vi "eDyno Accel Synth.vi"(0 "Fault Injection":T3={"Imbalance ON"=FALSE, "Imbalance (g)"=0.5, "Misalignment ON"=FALSE, "Misalignment (g)"=0.2, "Bearing BPFO ON"=FALSE, "Bearing Impact (g)"=2.0, "Motor Ripple ON"=FALSE, "Torque Ripple (g)"=0.3, "PWM Noise ON"=FALSE, "PWM Level (g)"=0.05}, 1 "Sim Config":T2={"Sample Rate (Hz)"=51200.0, "Ref Speed (rpm)"=3000.0, "Baseline 1x (g)"=0.02, "Noise Floor (g rms)"=0.01, "BPFO Order"=3.57, "Resonance (Hz)"=3500.0, "Decay (ms)"=0.8, "Pole Pairs"=4.0, "PWM Carrier (Hz)"=16000.0}, 2 "rpm start":dbl=3000.0, 3 "rpm end":dbl=3000.0, 4 "Samples":i32=5120, 5 "State in":cluster{"Shaft Rev":dbl, "Sample Index":dbl}) -> (14 "Accel (g)":dbl[](array[numeric]), 15 "Fault Frequencies (Hz)":T1, 16 "Speed (rpm)":dbl[](array[numeric]), 17 "Tach Pulse 1ppr (0/1)":dbl[](array[numeric]), 19 "State out":cluster{"Shaft Rev":dbl, "Sample Index":dbl})   [LabVIEW 2026]
doc: "Synthesizes one block of eDyno drivetrain acceleration (g) as seen by a PCB 356A15 ICP accelerometer (one axis) on an e-bike motor housing.\n\nSpeed ramps linearly from rpm start to rpm end across the block, and every order tracks speed. Shaft phase (revolutions) and the sample counter travel in State in/State out: feed State out back into State in through a shift register in the caller so consecutive blocks are phase-continuous.\n\nBaseline: a small 1x residual plus broadband noise. Injectable faults (Fault Injection cluster):\n- Imbalance: 1x order, amplitude scales with (rpm/ref)^2\n- Misalignment: 2x order\n- Bearing outer race (BPFO): impacts every 1/(BPFO order x shaft Hz) ringing the housing resonance with exponential decay\n- Motor torque ripple: 6 x pole-pairs order\n- Inverter PWM: carrier with sidebands at carrier +/- 2 x electrical frequency\n\nFault Frequencies returns the expected frequencies at rpm end, for the engineer to check against the spectrum. Speed (rpm) returns the instantaneous shaft speed per sample, and Tach Pulse 1ppr a 50 % duty once-per-rev square wave whose rising edge is at shaft angle 0 - both phase-locked to Accel (g) for order analysis."
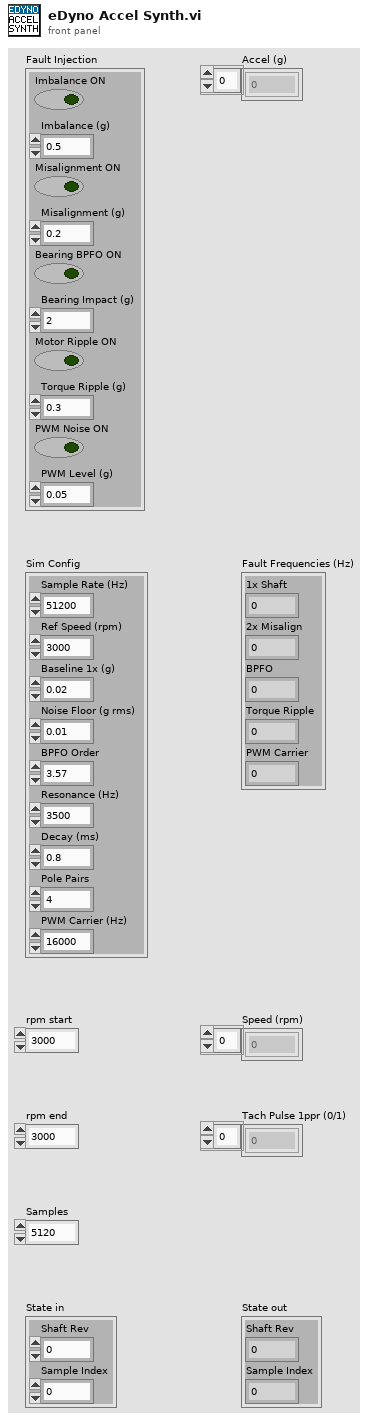
[diagram p1: front panel]
types:
  T1 = cluster{"1x Shaft":dbl, "2x Misalign":dbl, "BPFO":dbl, "Torque Ripple":dbl, "PWM Carrier":dbl}
  T2 = cluster{"Sample Rate (Hz)":dbl, "Ref Speed (rpm)":dbl, "Baseline 1x (g)":dbl, "Noise Floor (g rms)":dbl, "BPFO Order":dbl, "Resonance (Hz)":dbl, "Decay (ms)":dbl, "Pole Pairs":dbl, "PWM Carrier (Hz)":dbl}
  T3 = cluster{"Imbalance ON":bool, "Imbalance (g)":dbl, "Misalignment ON":bool, "Misalignment (g)":dbl, "Bearing BPFO ON":bool, "Bearing Impact (g)":dbl, "Motor Ripple ON":bool, "Torque Ripple (g)":dbl, "PWM Noise ON":bool, "PWM Level (g)":dbl}
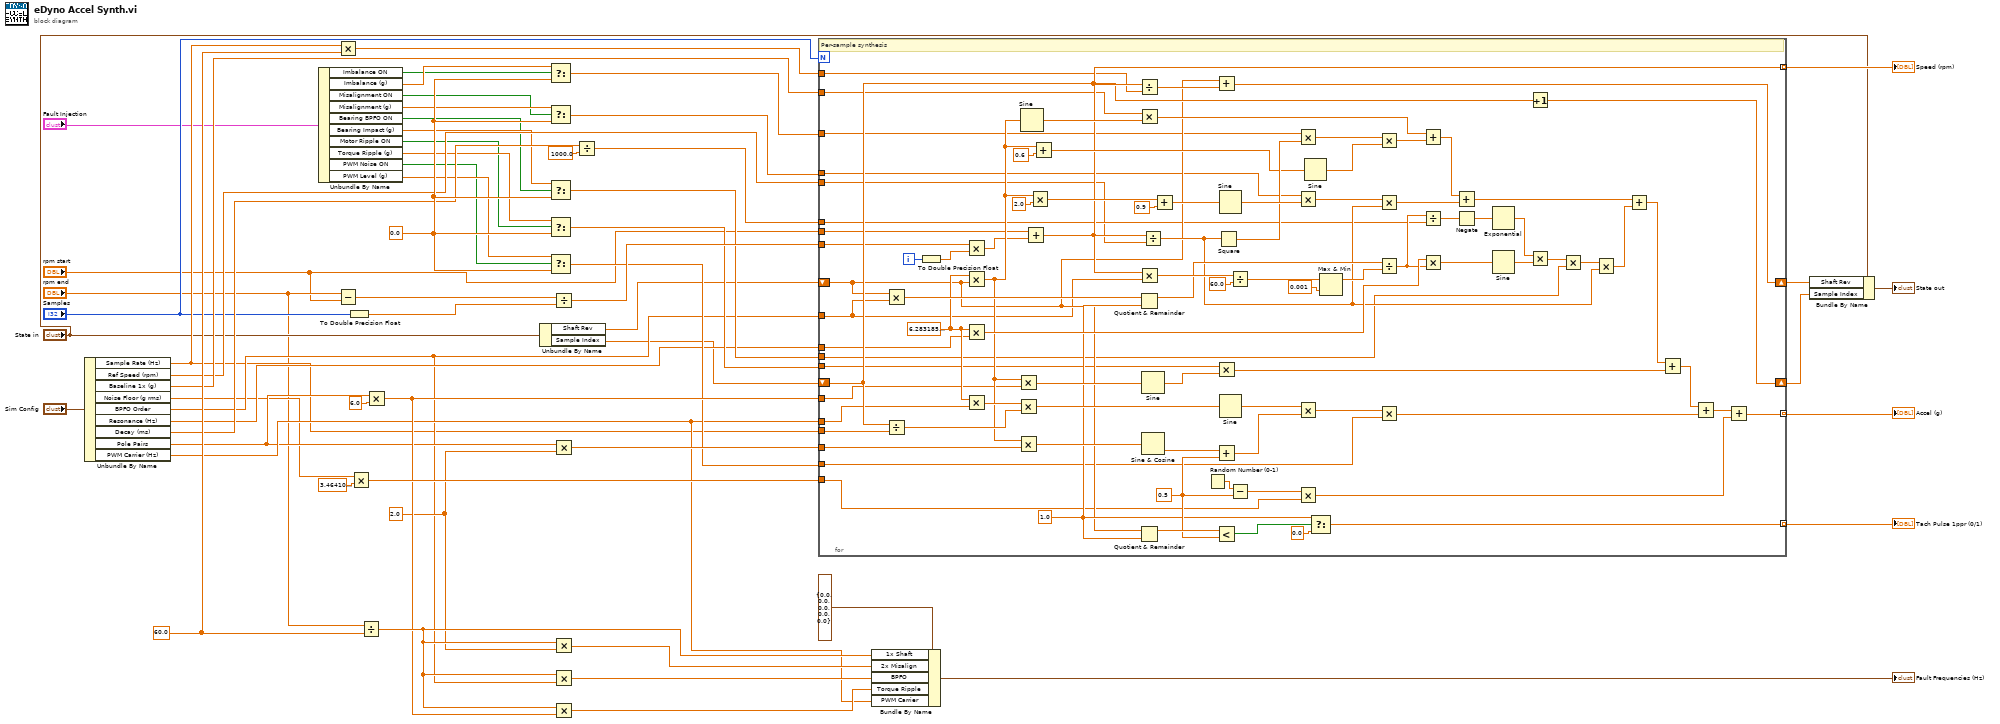
[diagram p0: block diagram]
diagram:
  w39 = 2.0 ("2")
  w36 = 60.0 ("60")
  w35 = 0.0 ("zero")
  n1 = Unbundle By Name("Sim Config") -> ("Sample Rate (Hz)"=w26:dbl, "Ref Speed (rpm)"=w27:dbl, "Baseline 1x (g)"=w28:dbl, "Noise Floor (g rms)"=w29:dbl, "BPFO Order"=w30:dbl, "Resonance (Hz)"=w31:dbl, "Decay (ms)"=w32:dbl, "Pole Pairs"=w33:dbl, "PWM Carrier (Hz)"=w34:dbl)
  n2 = Unbundle By Name("Fault Injection") -> ("Imbalance ON"=w16:bool, "Imbalance (g)"=w17:dbl, "Misalignment ON"=w18:bool, "Misalignment (g)"=w19:dbl, "Bearing BPFO ON"=w20:bool, "Bearing Impact (g)"=w21:dbl, "Motor Ripple ON"=w22:bool, "Torque Ripple (g)"=w23:dbl, "PWM Noise ON"=w24:bool, "PWM Level (g)"=w25:dbl)
  n3 = Multiply(x=w26, y=w36) -> (x*y=w49:dbl)
  n4 = Subtract(x="rpm end", y="rpm start") -> (x-y=w47:dbl)
  n5 = To Double Precision Float(number="Samples") -> (double precision float=w46:dbl)
  n6 = Multiply(x=w29, y=3.4641016151377544 ("sqrt12")) -> (x*y=w53:dbl)
  n7 = Divide(x="rpm end", y=w36) -> (x/y=w54:dbl)
  n8 = Multiply(x=w33, y=6.0 ("6")) -> (x*y=w51:dbl)
  n9 = Unbundle By Name("State in") -> ("Shaft Rev"=w12:dbl, "Sample Index"=w13:dbl)
  n10 = Select(t=w17, s=w16, f=w35) -> (s? t:f=w41:dbl)
  n11 = Select(t=w19, s=w18, f=w35) -> (s? t:f=w42:dbl)
  n12 = Select(t=w21, s=w20, f=w35) -> (s? t:f=w43:dbl)
  n13 = Select(t=w23, s=w22, f=w35) -> (s? t:f=w44:dbl)
  n14 = Select(t=w25, s=w24, f=w35) -> (s? t:f=w45:dbl)
  n15 = Divide(x=w47, y=w46) -> (x/y=w48:dbl)
  n16 = Multiply(x=w33, y=w39) -> (x*y=w52:dbl)
  n17 = Multiply(x=w54, y=w39) -> (x*y=w55:dbl)
  n18 = Multiply(x=w54, y=w30) -> (x*y=w56:dbl)
  n19 = Multiply(x=w54, y=w51) -> (x*y=w57:dbl)
  n20 = Divide(x=w32, y=1000.0 ("1000")) -> (x/y=w50:dbl)
  n21 = for {
    N: "Samples" -> [_]
    tunnel: "rpm start" -> [w60]
    tunnel: w26 -> [w63]
    tunnel: w27 -> [w64]
    tunnel: w28 -> [w65]
    tunnel: w30 -> [w68]
    tunnel: w31 -> [w70]
    tunnel: w34 -> [w74]
    shift-right: [w79] -> w14
    shift-left: w12 -> [w78]
    shift-right: [w81] -> w15
    shift-left: w13 -> [w80]
    tunnel: w48 -> [w61]
    tunnel: w49 -> [w62]
    tunnel: w41 -> [w66]
    tunnel: w42 -> [w67]
    tunnel: w50 -> [w69]
    tunnel: w43 -> [w71]
    tunnel: w51 -> [w72]
    tunnel: w44 -> [w73]
    tunnel: w52 -> [w75]
    tunnel: w45 -> [w76]
    tunnel: w53 -> [w77]
    tunnel: [w92] -> w10 mode=indexing
    tunnel: [w147] -> w11 mode=indexing
    tunnel: [w143] -> w6 mode=indexing
    i -> [w59]
    w89 = 0.5 ("half")
    w83 = 1.0 ("one")
    w82 = 6.283185307179586 ("2pi")
    # "Per-sample synthesis"
    n22 = Multiply(x=w78, y=w68) -> (x*y=w109:dbl)
    n23 = Divide(x=w80, y=w63) -> (x/y=w96:dbl)
    n24 = To Double Precision Float(number=w59) -> (double precision float=w90:dbl)
    n25 = Multiply(x=w61, y=w90) -> (x*y=w91:dbl)
    n26 = Multiply(x=w82, y=w78) -> (x*y=w94:dbl)
    n27 = Multiply(x=w82, y=w70) -> (x*y=w118:dbl)
    n28 = Multiply(x=w82, y=w74) -> (x*y=w127:dbl)
    n29 = Multiply(x=w94, y=w72) -> (x*y=w124:dbl)
    n30 = Multiply(x=w127, y=w96) -> (x*y=w128:dbl)
    n31 = Multiply(x=w94, y=w75) -> (x*y=w130:dbl)
    n32 = Sine(x=w94) -> (sin(x)=w97:dbl)
    n33 = Add(x=w60, y=w91) -> (x+y=w92:dbl)
    n34 = Multiply(x=w94, y=2.0 ("two")) -> (x*y=w104:dbl)
    n35 = Add(x=w94, y=0.6 ("imb phase")) -> (x+y=w99:dbl)
    n36 = Divide(x=w92, y=w62) -> (x/y=w93:dbl)
    n37 = Multiply(x=w65, y=w97) -> (x*y=w98:dbl)
    n38 = Multiply(x=w92, y=w68) -> (x*y=w111:dbl)
    n39 = Quotient & Remainder(x=w109, y=w83) -> (x-y*floor(x/y)=w110:dbl)  [unwired: 1 out]
    n40 = Quotient & Remainder(x=w78, y=w83) -> (x-y*floor(x/y)=w145:dbl)  [unwired: 1 out]
    n41 = Divide(x=w92, y=w64) -> (x/y=w95:dbl)
    n42 = Sine(x=w124) -> (sin(x)=w125:dbl)
    n43 = Sine & Cosine(0:w130) -> (2:w131:dbl)  [unwired: 1 out]
    n44 = Add(x=w104, y=0.9 ("mis phase")) -> (x+y=w105:dbl)
    n45 = Random Number (0-1)() -> (number: 0 to 1=w135:dbl)
    n46 = Add(x=w78, y=w93) -> (x+y=w79:dbl)
    n47 = Multiply(x=w73, y=w125) -> (x*y=w126:dbl)
    n48 = Add(x=w131, y=w89) -> (x+y=w132:dbl)
    n49 = Less?(x=w145, y=w89) -> (x < y?=w146:bool)
    n50 = Square(x=w95) -> (x^2=w101:dbl)
    n51 = Sine(x=w105) -> (sin(x)=w106:dbl)
    n52 = Sine(x=w128) -> (sin(x)=w129:dbl)
    n53 = Divide(x=w111, y=60.0 ("sixty")) -> (x/y=w112:dbl)
    n54 = Subtract(x=w135, y=w89) -> (x-y=w136:dbl)
    n55 = Multiply(x=w66, y=w101) -> (x*y=w102:dbl)
    n56 = Multiply(x=w67, y=w106) -> (x*y=w107:dbl)
    n57 = Multiply(x=w129, y=w132) -> (x*y=w133:dbl)
    n58 = Multiply(x=w136, y=w77) -> (x*y=w137:dbl)
    n59 = Sine(x=w99) -> (sin(x)=w100:dbl)
    n60 = Select(t=w83, s=w146, f=0.0 ("zero")) -> (s? t:f=w147:dbl)
    n61 = Max & Min(x=w112, y=0.001 ("min fB")) -> (max(x,y)=w113:dbl)  [unwired: 1 out]
    n62 = Multiply(x=w102, y=w100) -> (x*y=w103:dbl)
    n63 = Multiply(x=w107, y=w95) -> (x*y=w108:dbl)
    n64 = Divide(x=w110, y=w113) -> (x/y=w114:dbl)
    n65 = Multiply(x=w133, y=w76) -> (x*y=w134:dbl)
    n66 = Add(x=w98, y=w103) -> (x+y=w138:dbl)
    n67 = Divide(x=w114, y=w69) -> (x/y=w115:dbl)
    n68 = Multiply(x=w118, y=w114) -> (x*y=w119:dbl)
    n69 = Add(x=w138, y=w108) -> (x+y=w139:dbl)
    n70 = Negate(x=w115) -> (-x=w116:dbl)
    n71 = Exponential(1:w116) -> (0:w117:dbl)
    n72 = Sine(x=w119) -> (sin(x)=w120:dbl)
    n73 = Increment(x=w80) -> (x+1=w81:dbl)
    n74 = Multiply(x=w117, y=w120) -> (x*y=w121:dbl)
    n75 = Multiply(x=w121, y=w71) -> (x*y=w122:dbl)
    n76 = Multiply(x=w122, y=w95) -> (x*y=w123:dbl)
    n77 = Add(x=w139, y=w123) -> (x+y=w140:dbl)
    n78 = Add(x=w140, y=w126) -> (x+y=w141:dbl)
    n79 = Add(x=w141, y=w134) -> (x+y=w142:dbl)
    n80 = Add(x=w142, y=w137) -> (x+y=w143:dbl)
  }
  "Accel (g)" <- w6
  "Speed (rpm)" <- w10
  "Tach Pulse 1ppr (0/1)" <- w11
  n81 = Bundle By Name(cluster=T1 {"1x Shaft"=0.0, "2x Misalign"=0.0, "BPFO"=0.0, "Torque Ripple"=0.0, "PWM Carrier"=0.0} ("freq template"), "1x Shaft"=w54, "2x Misalign"=w55, "BPFO"=w56, "Torque Ripple"=w57, "PWM Carrier"=w34) -> (→"Fault Frequencies (Hz)":T1)
  n82 = Bundle By Name(cluster="State in", "Shaft Rev"=w14, "Sample Index"=w15) -> (→"State out":cluster{"Shaft Rev":dbl, "Sample Index":dbl})
